vi "ThermoelectricMeasureMain.vi"() -> ()   [LabVIEW 2024]
uses:
  <vilib>/MakerHub/LINX/LMH-LINX.lvlib
  Globals.vi
  <vilib>/addons/control/pid/NI_PID_pid.lvlib
  <vilib>/MakerHub/LINX/Public/Peripherals/PWM/PWM Set Duty Cycle 1 Chan.vi
  <vilib>/addons/control/pid/pid.llb/PID (DBL).vi
  <vilib>/Analysis/NI_AALBase.lvlib
  <vilib>/Utility/file.llb/Write Delimited Spreadsheet (string).vi
  <vilib>/MakerHub/LINX/Public/Peripherals/PWM/PWM Set Duty Cycle N Chans.vi
  <vilib>/MakerHub/LINX/Public/Peripherals/Analog/Analog Read N Chans.vi
  <vilib>/MakerHub/LINX/Public/Peripherals/Digital/Digital Read 1 Chan.vi
  <vilib>/MakerHub/LINX/Public/Utilities/Open Serial.vi
panel:
  in  "File Name":string
  in  "Save Folder":path
  out "A5":dbl
  out "Resistance Amplified":dbl
  out "Resistance A3":dbl
  in  "Current":dbl
  out "A2 (TH)":dbl
  out "A1 (Voltage)":dbl
  out "A0 (TC)":dbl
  out "Resistance Amplified":dbl(graph)
  out "A4":dbl
  out "A3":dbl
  out "Resistance A3":dbl(graph)
  out "TREF 2 Error":dbl
  out "TREF 2":dbl
  out "TREF 1 Error":dbl
  out "Seebeck Coeff":dbl
  out "TREF 1":dbl
  in  "Target TC":dbl format="%.2f"
  in  "Target TH":dbl format="%.2f"
  out "Auto":bool
  in  "Start Auto":bool
  in  "TH End":dbl(knob)=100.0 step=10.0 scale=0.0..100.0
  in  "TH Start":dbl(knob)=40.0 step=10.0 scale=0.0..100.0
  out "VOUT - 1.25":dbl(knob) scale=-1.0..1.0
  out "TC":dbl(slide) scale=0.0..100.0
  out "TH":dbl(slide) scale=0.0..100.0
  out "Voltage":dbl(graph)
  out "TH":dbl(graph)
  in  "Save to File":bool
  out "VOUT - 1.25":dbl
  out "TC":dbl(graph)
  out "TC":dbl
  in  "Stop Button":bool
  out "TH":dbl
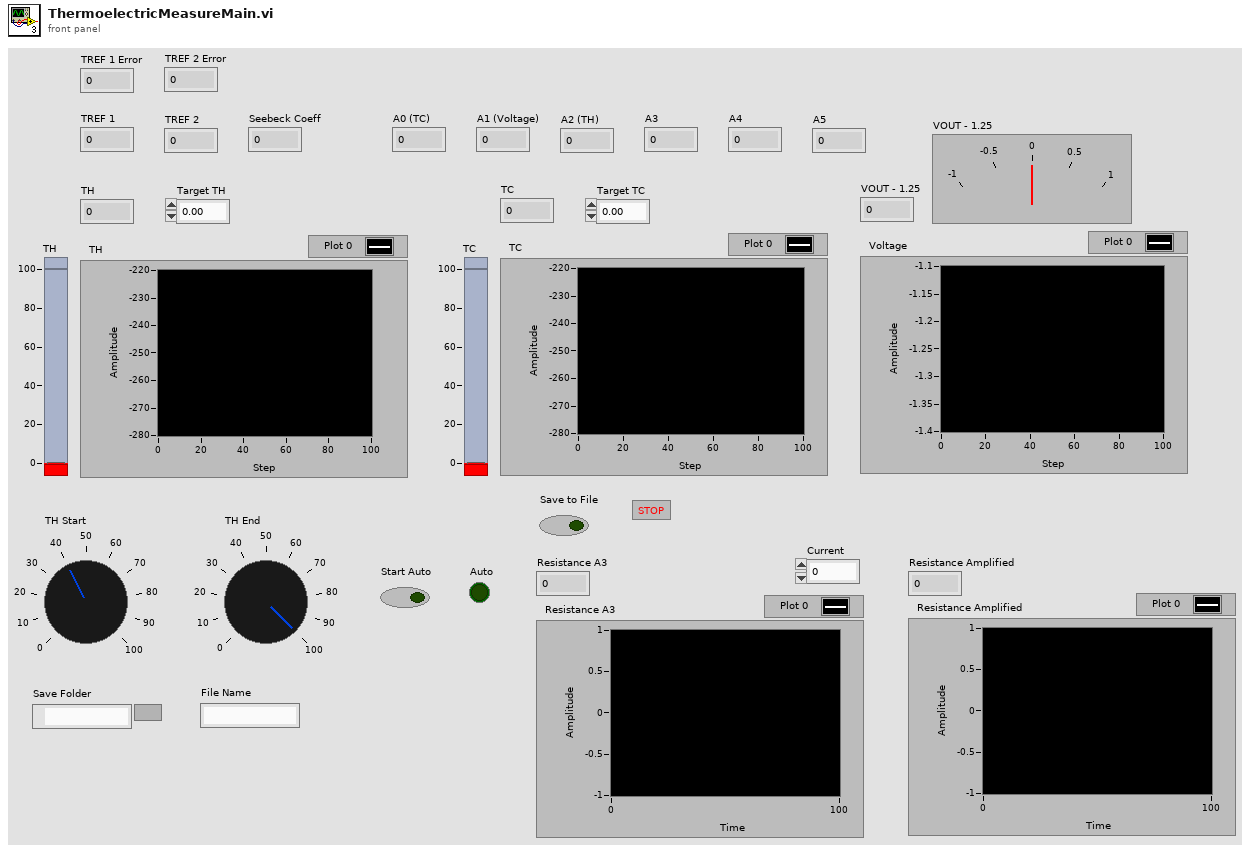
[diagram p1: front panel]
types:
  T1 = typedef "LMH-LINX.lvlib/LINX Ref.ctl" = cluster{"IO":T2, "Interface":T3, "LINX Device Config":T4}
  T2 = typedef "LMH-LINX.lvlib/Platform.ctl" = enum16{"Remote", "Local"}
  T3 = typedef "LMH-LINX.lvlib/Interface.ctl" = enum16{"Serial", "TCP"}
  T4 = typedef "LMH-LINX.lvlib/Device.lvlib/LINX Device Config.ctl" = cluster{"Interface":T3, "COM Port":refnum<visa-resource-name>, "TCP Configuration":T5, "Device Family":u8, "Device ID":u8, "Device Name":string, "TCP Ref":refnum<k5>, "Channels":T6}
  T5 = typedef "LMH-LINX.lvlib/Device.lvlib/TCP Config.ctl" = cluster{"IP Address":string, "Port":u16}
  T6 = typedef "LMH-LINX.lvlib/Channels.ctl" = cluster{"DI":u8[], "DO":u8[], "AI":u8[], "AO":u8[], "PWM":u8[], "QE":u8[], "UART":u8[], "I2C 2":u8[], "SPI":u8[], "CAN":u8[], "Servo":u8[], "AI Ref (V)":dbl, "AI Resolution (Bits)":u8, "AO Ref (V)":dbl, "AO Resolution (Bits)":u8}
  T7 = cluster{"proportional gain (Kc)":dbl, "integral time (Ti, min)":dbl, "derivative time (Td, min)":dbl}
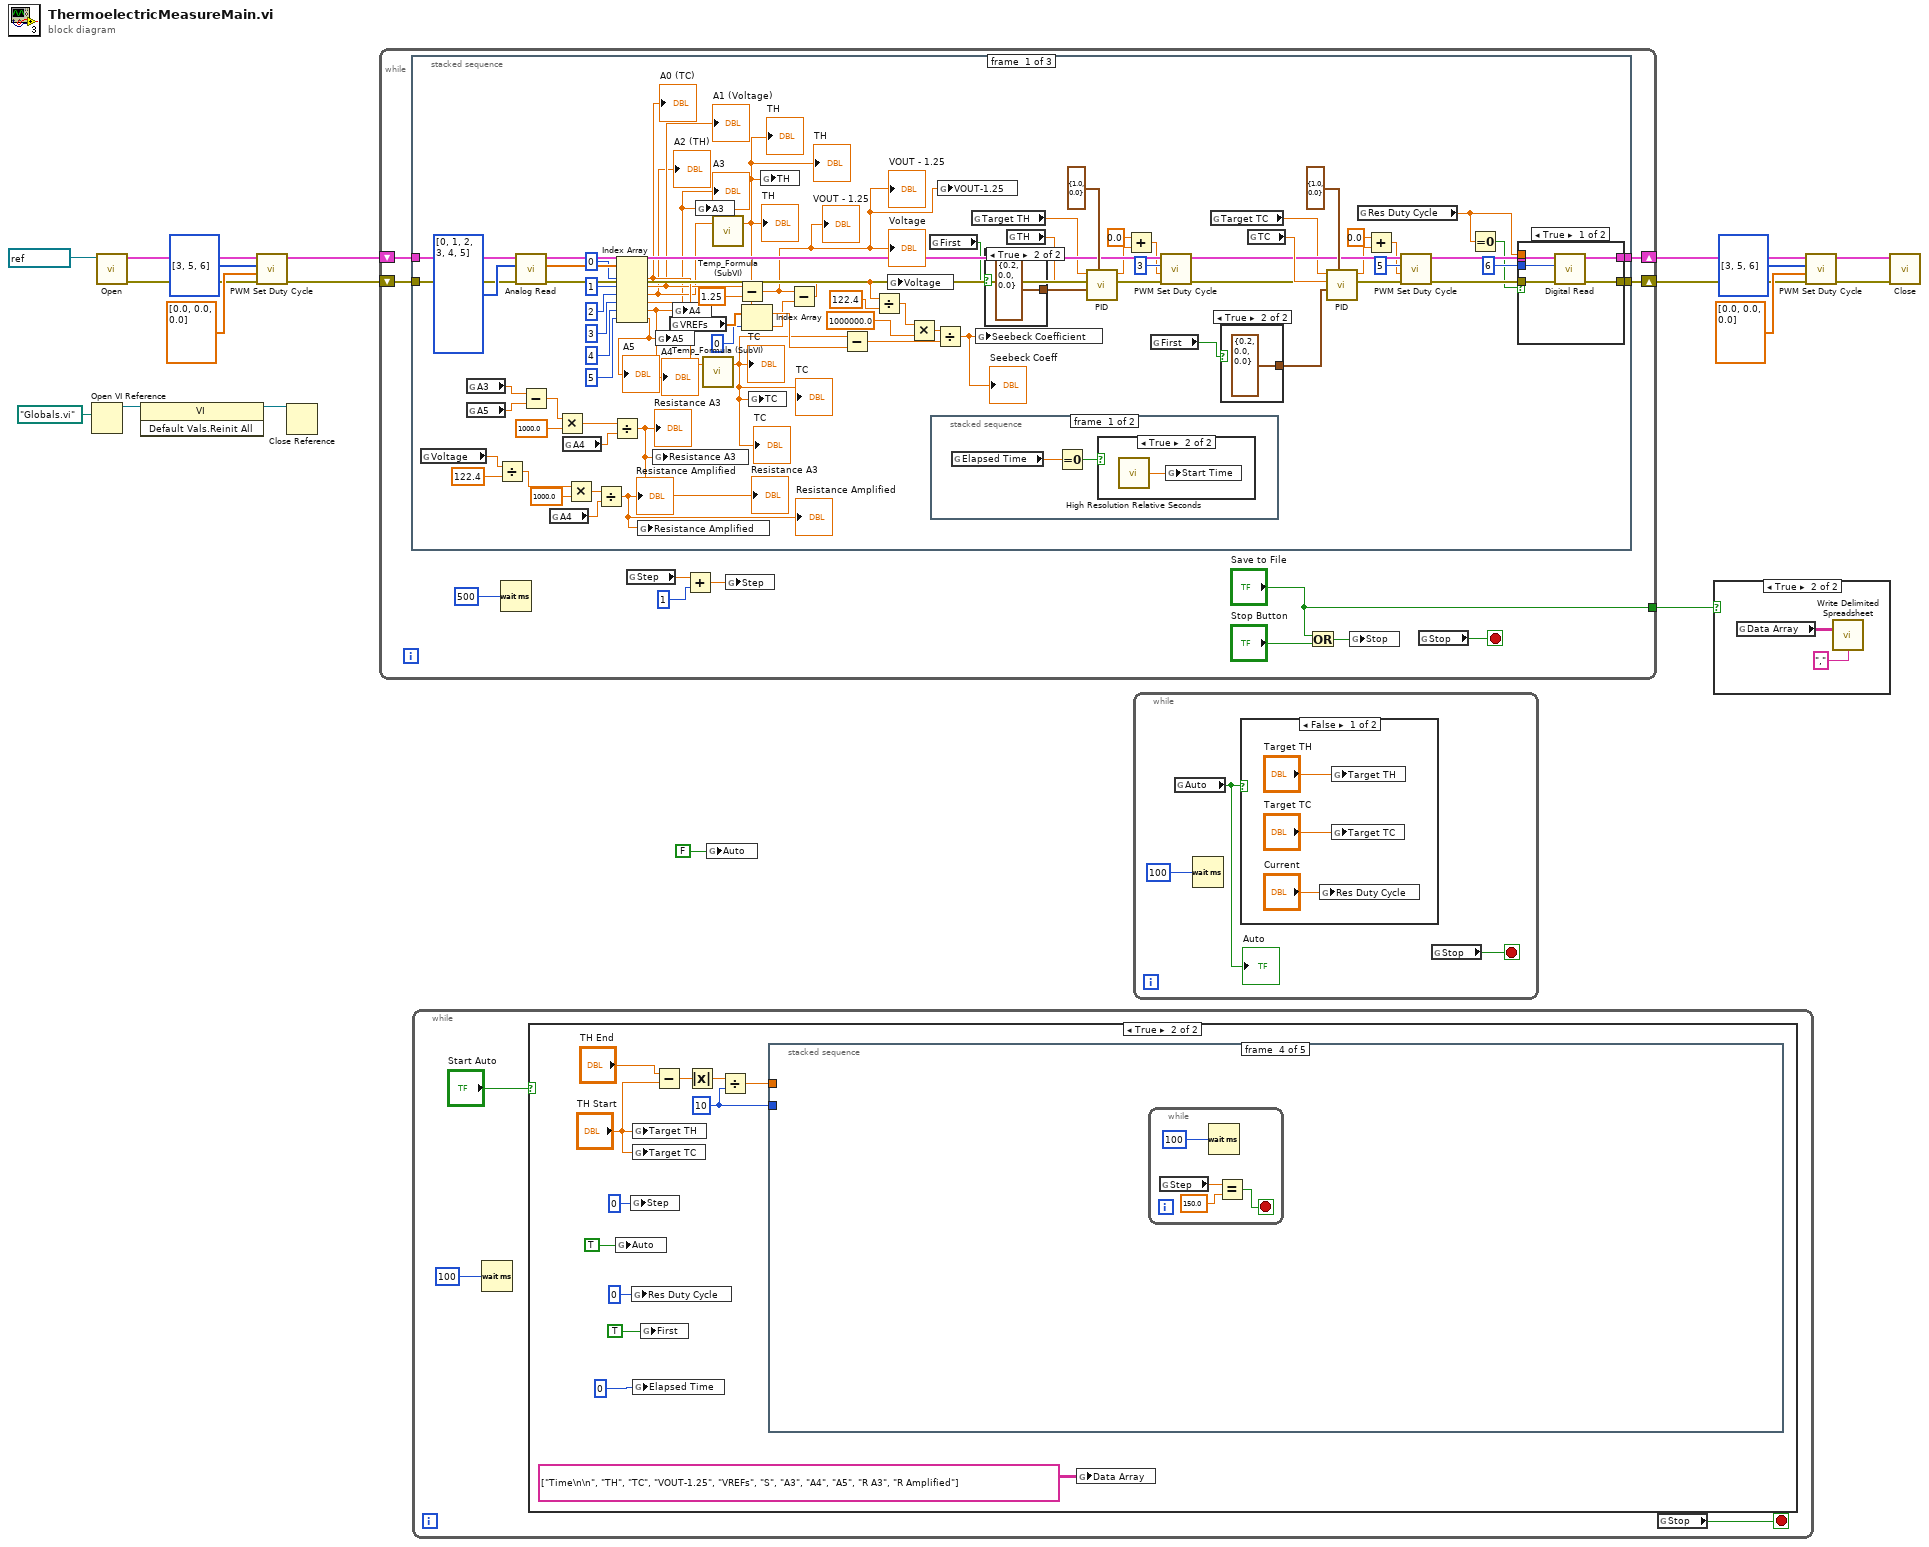
[diagram p0: block diagram]
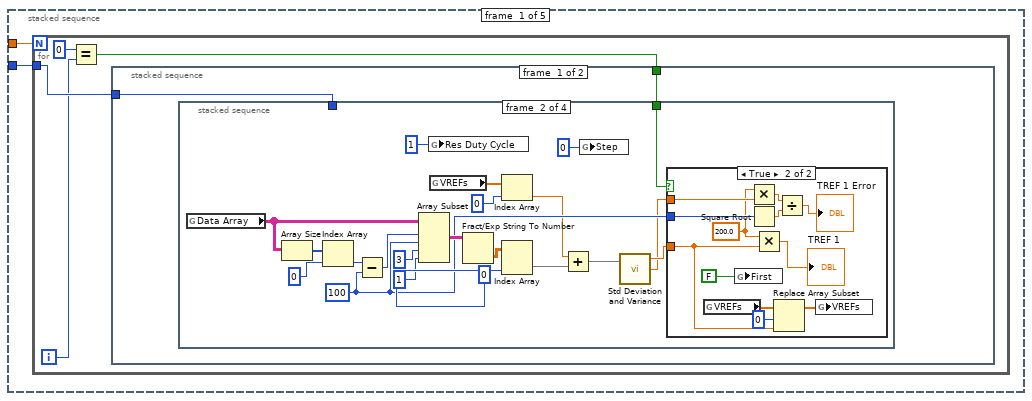
[diagram p3: hidden frame]
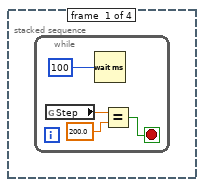
[diagram p4: hidden frame]
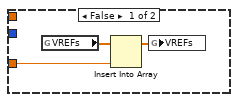
[diagram p5: hidden frame]
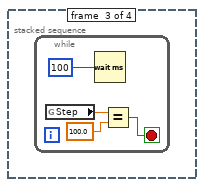
[diagram p6: hidden frame]
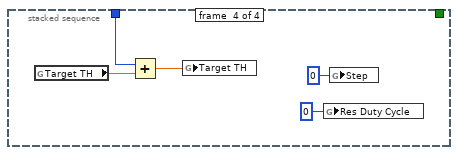
[diagram p7: hidden frame]
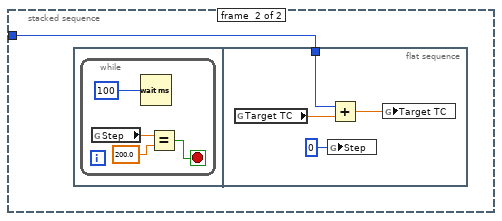
[diagram p8: hidden frame]
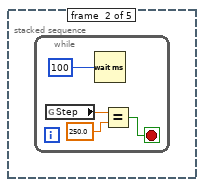
[diagram p9: hidden frame]
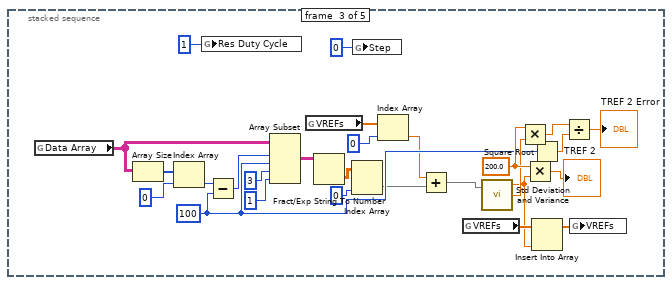
[diagram p10: hidden frame]
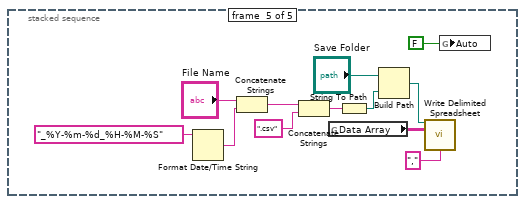
[diagram p11: hidden frame]
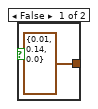
[diagram p14: hidden frame]
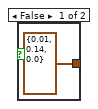
[diagram p15: hidden frame]
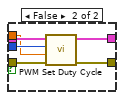
[diagram p16: hidden frame]
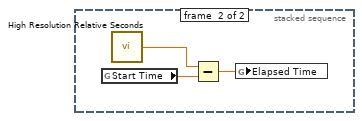
[diagram p18: hidden frame]
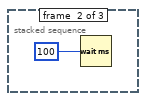
[diagram p19: hidden frame]
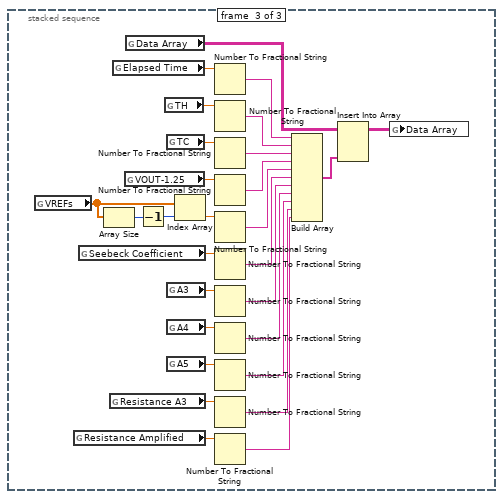
[diagram p20: hidden frame]
diagram:
  n1 = Open VI Reference(vi path=path "Globals.vi") -> (vi reference=w16:refnum<vi>)  [unwired: 5 in, 1 out]
  n2 = call-poly <vilib>:"Open.vi"("Serial Port"=refnum<visa-resource-name> "COM3") -> ("Error Out"=w8:errorcluster, "LINX Resource"=w11:T1)  [unwired: 8 in, 1 out]
  n3 = invoke class="VI" method="Default Vals.Reinit All"(reference=w16) -> (reference out=w15:refnum<vi>)  [unwired: 2 in, 2 out]
  n4 = call-poly <vilib>:"PWM Set Duty Cycle.vi"("Error In"=w8, "Duty Cycles"=dbl[] [0.0, 0.0, 0.0] ("Duty Cycle (0-1)"), "PWM Channels"=u8[] [3, 5, 6] ("PWM Channel"), "LINX Resource"=w11) -> ("Error Out"=w7:errorcluster, "LINX Resource"=w12:T1)  [unwired: 6 in]
  n5 = Close Reference(reference=w15) -> ()  [unwired: 1 in, 1 out]
  n6 = while {
    shift-right: [w29] -> w4
    shift-left: w12 -> [w30]
    shift-right: [w27] -> w1
    shift-left: w7 -> [w28]
    tunnel: ["Save to File"] -> w17
    stop <- w22 stop-if-true
    n7 = stacked-sequence {
      tunnel: w30 -> [w94 _ _]
      tunnel: [w62 _ _] -> w29
      tunnel: w28 -> [w93 _ _]
      tunnel: [w60 _ _] -> w27
      frame #0 {
        n8 = global read "Globals.vi" "Voltage"() -> (w58:dbl)
        n9 = global read "Globals.vi" "A3"() -> (w41:dbl)
        n10 = global read "Globals.vi" "A5"() -> (w47:dbl)
        n11 = Divide(x=w58, y=122.4) -> (x/y=w44:dbl)
        n12 = call-poly <vilib>:"Analog Read.vi"("Error In"=w93, "AI Channel(s)"=i32[] [0, 1, 2, 3, 4, 5], "LINX Resource"=w94) -> ("Error Out"=w91:errorcluster, "Voltages"=w100:dbl[], "LINX Resource"=w92:T1)  [unwired: 5 in, 1 out]
        n13 = Subtract(x=w41, y=w47) -> (x-y=w45:dbl)
        n14 = global read "Globals.vi" "A4"() -> (w33:dbl)
        n15 = Multiply(x=w45, y=1000.0) -> (x*y=w71:dbl)
        n16 = global read "Globals.vi" "A4"() -> (w34:dbl)
        n17 = Multiply(x=w44, y=1000.0) -> (x*y=w67:dbl)
        n18 = Divide(x=w67, y=w33) -> (x/y=w56:dbl)
        "Resistance Amplified" <- w56
        "Resistance Amplified" <- w56
        n19 = Divide(x=w71, y=w34) -> (x/y=w57:dbl)
        "Resistance A3" <- w57
        "Resistance A3" <- w57
        n20 = Index Array(array=w100, index #1=0 ("index"), index #2=1 ("index"), index #3=2 ("index"), index #4=3 ("index"), index #5=4 ("index"), index #6=5 ("index")) -> (element #1=w66:dbl, element #2=w65:dbl, element #3=w64:dbl, element #4=w54:dbl, element #5=w53:dbl, element #6=w49:dbl)
        "A3" <- w54
        "A4" <- w53
        "A0 (TC)" <- w66
        "A1 (Voltage)" <- w65
        "A2 (TH)" <- w64
        "A5" <- w49
        n21 = global write "Globals.vi" "Resistance Amplified"(w56) -> ()
        n22 = global write "Globals.vi" "Resistance A3"(w57) -> ()
        n23 = global write "Globals.vi" "A5"(w49) -> ()
        n24 = global read "Globals.vi" "VREFs"() -> (w75:dbl[])
        n25 = global write "Globals.vi" "A4"(w53) -> ()
        n26 = global write "Globals.vi" "A3"(w54) -> ()
        n27 = call "Temp_Formula (SubVI).vi"("In"=w66) -> ("Out"=w76:dbl)  [unwired: 1 in, 1 out]
        "TC" <- w76
        "TC" <- w76
        "TC" <- w76
        n28 = call "Temp_Formula (SubVI).vi"("In"=w64) -> ("Out"=w77:dbl)  [unwired: 1 in, 1 out]
        "TH" <- w77
        "TH" <- w77
        "TH" <- w77
        n29 = Subtract(x=w65, y=1.25) -> (x-y=w55:dbl)
        "VOUT - 1.25" <- w55
        "Voltage" <- w55
        "VOUT - 1.25" <- w55
        n30 = Index Array(array=w75, index=0) -> (element=w73:dbl)
        n31 = global write "Globals.vi" "TC"(w76) -> ()
        n32 = global write "Globals.vi" "TH"(w77) -> ()
        n33 = Subtract(x=w55, y=w73) -> (x-y=w72:dbl)
        n34 = Subtract(x=w76, y=w77) -> (x-y=w103:dbl)
        n35 = Divide(x=w72, y=122.4) -> (x/y=w78:dbl)
        n36 = global write "Globals.vi" "Voltage"(w72) -> ()
        n37 = Multiply(x=w78, y=1000000.0) -> (x*y=w81:dbl)
        n38 = global read "Globals.vi" "First"() -> (w43:bool)
        n39 = stacked-sequence {
          frame #0 {
            n40 = global read "Globals.vi" "Elapsed Time"() -> (w119:dbl)
            n41 = Equal To 0?(x=w119) -> (x = 0?=w120:bool)
            n42 = case shown="True" w120 {
              frame False {
              }
              frame True {
                n43 = call <vilib>:"High Resolution Relative Seconds.vi"() -> ("relative seconds"=w121:dbl)
                n44 = global write "Globals.vi" "Start Time"(w121) -> ()
              }
            }
          }
          frame #1 {
            n45 = global read "Globals.vi" "Start Time"() -> (w122:dbl)
            n46 = call <vilib>:"High Resolution Relative Seconds.vi"() -> ("relative seconds"=w123:dbl)
            n47 = Subtract(x=w123, y=w122) -> (x-y=w124:dbl)
            n48 = global write "Globals.vi" "Elapsed Time"(w124) -> ()
          }
        }
        n49 = Divide(x=w81, y=w103) -> (x/y=w102:dbl)
        "Seebeck Coeff" <- w102
        n50 = global write "Globals.vi" "VOUT-1.25"(w55) -> ()
        n51 = global read "Globals.vi" "Target TH"() -> (w84:dbl)
        n52 = global write "Globals.vi" "Seebeck Coefficient"(w102) -> ()
        n53 = case shown="True" w43 {
          tunnel: [T7 {"proportional gain (Kc)"=0.01, "integral time (Ti, min)"=0.14, "derivative time (Td, min)"=0.0} ("PID gains") T7 {"proportional gain (Kc)"=0.2, "integral time (Ti, min)"=0.0, "derivative time (Td, min)"=0.0} ("PID gains")] -> w42
          frame False {
          }
          frame True {
          }
        }
        n54 = global read "Globals.vi" "TH"() -> (w90:dbl)
        n55 = call-poly <vilib>:"PID.vi"("output range"=cluster{"output high":dbl, "output low":dbl} {"output high"=1.0, "output low"=0.0}, "PID gains"=w42, "process variable"=w90, "setpoint"=w84) -> ("output"=w37:dbl)  [unwired: 6 in, 1 out]
        n56 = Add(x=0.0, y=w37) -> (x+y=w36:dbl)
        n57 = global read "Globals.vi" "First"() -> (w32:bool)
        n58 = call-poly <vilib>:"PWM Set Duty Cycle.vi"("Error In"=w91, "Duty Cycle (0-1)"=w36, "PWM Channel"=u8 3, "LINX Resource"=w92) -> ("Error Out"=w85:errorcluster, "LINX Resource"=w86:T1)  [unwired: 6 in]
        n59 = global read "Globals.vi" "Target TC"() -> (w83:dbl)
        n60 = case shown="True" w32 {
          tunnel: [T7 {"proportional gain (Kc)"=0.01, "integral time (Ti, min)"=0.14, "derivative time (Td, min)"=0.0} ("PID gains") T7 {"proportional gain (Kc)"=0.2, "integral time (Ti, min)"=0.0, "derivative time (Td, min)"=0.0} ("PID gains")] -> w31
          frame False {
          }
          frame True {
          }
        }
        n61 = global read "Globals.vi" "TC"() -> (w87:dbl)
        n62 = call-poly <vilib>:"PID.vi"("output range"=cluster{"output high":dbl, "output low":dbl} {"output high"=1.0, "output low"=0.0}, "PID gains"=w31, "process variable"=w87, "setpoint"=w83) -> ("output"=w40:dbl)  [unwired: 6 in, 1 out]
        n63 = global read "Globals.vi" "Res Duty Cycle"() -> (w52:dbl)
        n64 = Add(x=0.0, y=w40) -> (x+y=w39:dbl)
        n65 = call-poly <vilib>:"PWM Set Duty Cycle.vi"("Error In"=w85, "Duty Cycle (0-1)"=w39, "PWM Channel"=u8 5, "LINX Resource"=w86) -> ("Error Out"=w61:errorcluster, "LINX Resource"=w63:T1)  [unwired: 6 in]
        n66 = Equal To 0?(x=w52) -> (x = 0?=w51:bool)
        n67 = case shown="True" w51 {
          tunnel: w63 -> [w112 w118]
          tunnel: [w111 w117] -> w62
          tunnel: w61 -> [w109 w116]
          tunnel: [w110 w115] -> w60
          tunnel: u8 6 ("PWM Channel") -> [w108 w114]
          tunnel: w52 -> [_ w113]
          frame True {
            n68 = call-poly <vilib>:"Digital Read.vi"("Error In"=w109, "DI Channel"=w108, "LINX Resource"=w112) -> ("Error Out"=w110:errorcluster, "LINX Resource"=w111:T1)  [unwired: 6 in, 1 out]
          }
          frame False {
            n69 = call-poly <vilib>:"PWM Set Duty Cycle.vi"("Error In"=w116, "Duty Cycle (0-1)"=w113, "PWM Channel"=w114, "LINX Resource"=w118) -> ("Error Out"=w115:errorcluster, "LINX Resource"=w117:T1)  [unwired: 6 in]
          }
        }
      }
      frame #1 {
        n70 = Wait (ms)(milliseconds to wait=u32 100) -> ()  [unwired: 1 out]
      }
      frame #2 {
        n71 = global read "Globals.vi" "VREFs"() -> (w140:dbl[])
        n72 = global read "Globals.vi" "Resistance Amplified"() -> (w127:dbl)
        n73 = global read "Globals.vi" "Seebeck Coefficient"() -> (w144:dbl)
        n74 = Array Size(array=w140) -> (size(s)=w139:i32)
        n75 = global read "Globals.vi" "Resistance A3"() -> (w131:dbl)
        n76 = global read "Globals.vi" "Elapsed Time"() -> (w142:dbl)
        n77 = global read "Globals.vi" "VOUT-1.25"() -> (w149:dbl)
        n78 = global read "Globals.vi" "Data Array"() -> (w152:string[][])
        n79 = Decrement(x=w139) -> (x-1=w138:i32)
        n80 = global read "Globals.vi" "TH"() -> (w145:dbl)
        n81 = global read "Globals.vi" "TC"() -> (w147:dbl)
        n82 = global read "Globals.vi" "A3"() -> (w132:dbl)
        n83 = global read "Globals.vi" "A4"() -> (w133:dbl)
        n84 = global read "Globals.vi" "A5"() -> (w130:dbl)
        n85 = Index Array(array=w140, index=w138) -> (element=w137:dbl)
        n86 = Number To Fractional String(number=w142) -> (F-format string=w143:string)  [unwired: 3 in]
        n87 = Number To Fractional String(number=w145) -> (F-format string=w146:string)  [unwired: 3 in]
        n88 = Number To Fractional String(number=w147) -> (F-format string=w148:string)  [unwired: 3 in]
        n89 = Number To Fractional String(number=w149) -> (F-format string=w150:string)  [unwired: 3 in]
        n90 = Number To Fractional String(number=w137) -> (F-format string=w136:string)  [unwired: 3 in]
        n91 = Number To Fractional String(number=w144) -> (F-format string=w141:string)  [unwired: 3 in]
        n92 = Number To Fractional String(number=w132) -> (F-format string=w135:string)  [unwired: 3 in]
        n93 = Number To Fractional String(number=w133) -> (F-format string=w134:string)  [unwired: 3 in]
        n94 = Number To Fractional String(number=w130) -> (F-format string=w129:string)  [unwired: 3 in]
        n95 = Number To Fractional String(number=w131) -> (F-format string=w128:string)  [unwired: 3 in]
        n96 = Number To Fractional String(number=w127) -> (F-format string=w126:string)  [unwired: 3 in]
        n97 = Build Array(w143, w146, w148, w150, w136, w141, w135, w134, w129, w128, w126) -> (w151:string[])
        n98 = Insert Into Array(array=w152, new element=w151) -> (w153:string[][])  [unwired: 2 in]
        n99 = global write "Globals.vi" "Data Array"(w153) -> ()
      }
    }
    n100 = Wait (ms)(milliseconds to wait=u32 500) -> ()  [unwired: 1 out]
    n101 = global read "Globals.vi" "Step"() -> (w21:dbl)
    n102 = Add(x=w21, y=1) -> (x+y=w20:dbl)
    n103 = global write "Globals.vi" "Step"(w20) -> ()
    n104 = Or(x="Save to File", y="Stop Button") -> (x .or. y?=w23:bool)
    n105 = global write "Globals.vi" "Stop"(w23) -> ()
    n106 = global read "Globals.vi" "Stop"() -> (w22:bool)
  }
  n107 = while {
    stop <- w155 stop-if-true
    n108 = Wait (ms)(milliseconds to wait=u32 100) -> ()  [unwired: 1 out]
    n109 = case shown="True" "Start Auto" {
      frame False {
      }
      frame True {
        w163 = 10
        n110 = global write "Globals.vi" "Auto"(TRUE) -> ()
        n111 = global write "Globals.vi" "Step"(0) -> ()
        n112 = global write "Globals.vi" "Res Duty Cycle"(0) -> ()
        n113 = global write "Globals.vi" "Target TH"("TH Start") -> ()
        n114 = global write "Globals.vi" "Target TC"("TH Start") -> ()
        n115 = global write "Globals.vi" "Elapsed Time"(0) -> ()
        n116 = global write "Globals.vi" "First"(TRUE) -> ()
        n117 = Subtract(x="TH End", y="TH Start") -> (x-y=w166:dbl)
        n118 = Absolute Value(x=w166) -> (abs(x)=w165:dbl)
        n119 = Divide(x=w165, y=w163) -> (x/y=w162:dbl)
        n120 = stacked-sequence {
          tunnel: w162 -> [w170 _ _ _ _]
          tunnel: w163 -> [w169 _ _ _ _]
          frame #0 {
            n121 = for {
              N: w170 -> [_]
              tunnel: w169 -> [w174]
              i -> [w171]
              n122 = Equal?(x=0 ("y"), y=w171) -> (x = y?=w173:bool)
              n123 = stacked-sequence {
                tunnel: w174 -> [w176 w226]
                tunnel: w173 -> [w175 _]
                frame #0 {
                  n124 = stacked-sequence {
                    tunnel: w176 -> [_ _ _ w223]
                    tunnel: w175 -> [_ w201 _ _]
                    frame #0 {
                      n125 = while {
                        stop <- w177 stop-if-true
                        n126 = global read "Globals.vi" "Step"() -> (w179:dbl)
                        n127 = Wait (ms)(milliseconds to wait=u32 100) -> ()  [unwired: 1 out]
                        n128 = Equal?(x=w179, y=200.0) -> (x = y?=w177:bool)
                      }
                    }
                    frame #1 {
                      w189 = 100 ("y")
                      n129 = global read "Globals.vi" "Data Array"() -> (w195:string[][])
                      n130 = Array Size(array=w195) -> (size(s)=w196:i32[])
                      n131 = Index Array(array=w196, index=0) -> (element=w197:i32)
                      n132 = Subtract(x=w197, y=w189) -> (x-y=w198:i32)
                      n133 = Array Subset(array=w195, index (row)=w198, length (row)=w189, index (col)=3 ("index"), length (col)=1 ("length")) -> (w199:string[][])
                      n134 = global write "Globals.vi" "Res Duty Cycle"(1) -> ()
                      n135 = global read "Globals.vi" "VREFs"() -> (w187:dbl[])
                      n136 = Fract/Exp String To Number(string=w199) -> (number=w200:dbl[][])  [unwired: 3 in, 1 out]
                      n137 = Index Array(array=w187, index=0) -> (element=w185:dbl)
                      n138 = Index Array(array=w200, index (col)=0 ("dimension size")) -> (element=w183:dbl[])  [unwired: 1 in]
                      n139 = Add(x=w185, y=w183) -> (x+y=w184:dbl[])
                      n140 = global write "Globals.vi" "Step"(0) -> ()
                      n141 = call <vilib>:"Std Deviation and Variance.vi"("X"=w184) -> ("mean"=w190:dbl, "standard deviation"=w188:dbl)  [unwired: 1 in, 1 out]
                      n142 = case shown="True" w201 {
                        tunnel: w190 -> [w202 w207]
                        tunnel: w189 -> [_ w214]
                        tunnel: w188 -> [_ w213]
                        frame False {
                          n143 = global read "Globals.vi" "VREFs"() -> (w203:dbl[])
                          n144 = Insert Into Array(array=w203, new element=w202) -> (w204:dbl[])  [unwired: 1 in]
                          n145 = global write "Globals.vi" "VREFs"(w204) -> ()
                        }
                        frame True {
                          w210 = 200.0 ("x")
                          n146 = global read "Globals.vi" "VREFs"() -> (w209:dbl[])
                          n147 = global write "Globals.vi" "First"(FALSE) -> ()
                          n148 = Multiply(x=w210, y=w213) -> (x*y=w215:dbl)
                          n149 = Square Root(x=w214) -> (sqrt(x)=w211:dbl)
                          n150 = Multiply(x=w210, y=w207) -> (x*y=→"TREF 1":dbl)
                          n151 = Replace Array Subset(array=w209, new element=w207, index=0) -> (w208:dbl[])
                          n152 = Divide(x=w215, y=w211) -> (x/y=→"TREF 1 Error":dbl)
                          n153 = global write "Globals.vi" "VREFs"(w208) -> ()
                        }
                      }
                    }
                    frame #2 {
                      n154 = while {
                        stop <- w217 stop-if-true
                        n155 = global read "Globals.vi" "Step"() -> (w219:dbl)
                        n156 = Wait (ms)(milliseconds to wait=u32 100) -> ()  [unwired: 1 out]
                        n157 = Equal?(x=w219, y=100.0) -> (x = y?=w217:bool)
                      }
                    }
                    frame #3 {
                      n158 = global read "Globals.vi" "Target TH"() -> (w225:dbl)
                      n159 = Add(x=w223, y=w225) -> (x+y=w224:dbl)
                      n160 = global write "Globals.vi" "Target TH"(w224) -> ()
                      n161 = global write "Globals.vi" "Res Duty Cycle"(0) -> ()
                      n162 = global write "Globals.vi" "Step"(0) -> ()
                    }
                  }
                }
                frame #1 {
                  n163 = flat-sequence {
                    tunnel: w226 -> [w232]
                    frame #0 {
                      n164 = while {
                        stop <- w227 stop-if-true
                        n165 = global read "Globals.vi" "Step"() -> (w229:dbl)
                        n166 = Wait (ms)(milliseconds to wait=u32 100) -> ()  [unwired: 1 out]
                        n167 = Equal?(x=w229, y=200.0) -> (x = y?=w227:bool)
                      }
                    }
                    frame #1 {
                      n168 = global read "Globals.vi" "Target TC"() -> (w233:dbl)
                      n169 = global write "Globals.vi" "Step"(0) -> ()
                      n170 = Add(x=w232, y=w233) -> (x+y=w234:dbl)
                      n171 = global write "Globals.vi" "Target TC"(w234) -> ()
                    }
                  }
                }
              }
            }
          }
          frame #1 {
            n172 = while {
              stop <- w235 stop-if-true
              n173 = global read "Globals.vi" "Step"() -> (w237:dbl)
              n174 = Wait (ms)(milliseconds to wait=u32 100) -> ()  [unwired: 1 out]
              n175 = Equal?(x=w237, y=250.0) -> (x = y?=w235:bool)
            }
          }
          frame #2 {
            w256 = 200.0 ("x")
            w251 = 100 ("y")
            n176 = global read "Globals.vi" "Data Array"() -> (w265:string[][])
            n177 = Array Size(array=w265) -> (size(s)=w263:i32[])
            n178 = Index Array(array=w263, index=0) -> (element=w261:i32)
            n179 = global write "Globals.vi" "Res Duty Cycle"(1) -> ()
            n180 = Subtract(x=w261, y=w251) -> (x-y=w260:i32)
            n181 = Array Subset(array=w265, index (row)=w260, length (row)=w251, index (col)=3 ("index"), length (col)=1 ("length")) -> (w257:string[][])
            n182 = global read "Globals.vi" "VREFs"() -> (w245:dbl[])
            n183 = Fract/Exp String To Number(string=w257) -> (number=w250:dbl[][])  [unwired: 3 in, 1 out]
            n184 = Index Array(array=w250, index (col)=0 ("dimension size")) -> (element=w241:dbl[])  [unwired: 1 in]
            n185 = global write "Globals.vi" "Step"(0) -> ()
            n186 = Index Array(array=w245, index=0) -> (element=w243:dbl)
            n187 = Add(x=w243, y=w241) -> (x+y=w242:dbl[])
            n188 = global read "Globals.vi" "VREFs"() -> (w247:dbl[])
            n189 = call <vilib>:"Std Deviation and Variance.vi"("X"=w242) -> ("mean"=w246:dbl, "standard deviation"=w255:dbl)  [unwired: 1 in, 1 out]
            n190 = Multiply(x=w256, y=w255) -> (x*y=w254:dbl)
            n191 = Multiply(x=w256, y=w246) -> (x*y=→"TREF 2":dbl)
            n192 = Square Root(x=w251) -> (sqrt(x)=w253:dbl)
            n193 = Insert Into Array(array=w247, new element=w246) -> (w248:dbl[])  [unwired: 1 in]
            n194 = Divide(x=w254, y=w253) -> (x/y=→"TREF 2 Error":dbl)
            n195 = global write "Globals.vi" "VREFs"(w248) -> ()
          }
          frame #3 {
            n196 = while {
              stop <- w266 stop-if-true
              n197 = global read "Globals.vi" "Step"() -> (w268:dbl)
              n198 = Wait (ms)(milliseconds to wait=u32 100) -> ()  [unwired: 1 out]
              n199 = Equal?(x=w268, y=150.0) -> (x = y?=w266:bool)
            }
          }
          frame #4 {
            n200 = Format Date/Time String(time format string (%c)="_%Y-%m-%d_%H-%M-%S") -> (date/time string=w274:string)  [unwired: 2 in]
            n201 = Concatenate Strings("File Name", w274) -> (w273:string)
            n202 = Concatenate Strings(w273, ".csv" ("string")) -> (w272:string)
            n203 = global read "Globals.vi" "Data Array"() -> (w280:string[][])
            n204 = String To Path(string=w272) -> (path=w271:path)
            n205 = Build Path(base path="Save Folder", name or relative path=w271) -> (appended path=w270:path)
            n206 = call-poly <vilib>:"Write Delimited Spreadsheet.vi"("file path (dialog if empty)"=w270, "2D data"=w280, "delimiter (\\t)"="," ("delimiter (\\t)")) -> ()  [unwired: 11 in, 2 out]
            n207 = global write "Globals.vi" "Auto"(FALSE) -> ()
          }
        }
        n208 = global write "Globals.vi" "Data Array"(string[][] [["Time\n\n", "TH", "TC", "VOUT-1.25", "VREFs", "S", "A3", "A4", "A5", "R A3", "R Amplified"]]) -> ()
      }
    }
    n209 = global read "Globals.vi" "Stop"() -> (w155:bool)
  }
  n210 = global write "Globals.vi" "Auto"(FALSE) -> ()
  n211 = while {
    stop <- w283 stop-if-true
    n212 = global read "Globals.vi" "Auto"() -> (w284:bool)
    "Auto" <- w284
    n213 = Wait (ms)(milliseconds to wait=u32 100) -> ()  [unwired: 1 out]
    n214 = case shown="False" w284 {
      frame False {
        n215 = global write "Globals.vi" "Res Duty Cycle"("Current") -> ()
        n216 = global write "Globals.vi" "Target TH"("Target TH") -> ()
        n217 = global write "Globals.vi" "Target TC"("Target TC") -> ()
      }
      frame True {
      }
    }
    n218 = global read "Globals.vi" "Stop"() -> (w283:bool)
  }
  n219 = case shown="True" w17 {
    frame False {
    }
    frame True {
      n220 = global read "Globals.vi" "Data Array"() -> (w289:string[][])
      n221 = call-poly <vilib>:"Write Delimited Spreadsheet.vi"("2D data"=w289, "delimiter (\\t)"="," ("delimiter (\\t)")) -> ()  [unwired: 12 in, 2 out]
    }
  }
  n222 = call-poly <vilib>:"PWM Set Duty Cycle.vi"("Error In"=w1, "Duty Cycles"=dbl[] [0.0, 0.0, 0.0] ("Duty Cycle (0-1)"), "PWM Channels"=u8[] [3, 5, 6] ("PWM Channel"), "LINX Resource"=w4) -> ("Error Out"=w2:errorcluster, "LINX Resource"=w3:T1)  [unwired: 6 in]
  n223 = call <vilib>:"Close.vi"("Error In"=w2, "LINX Resource"=w3) -> ()  [unwired: 9 in, 1 out]
